vi "RemoteVI Accept Clients.vi"(0 "new connection":u32, 1 "html":string, 2 "hello":string, 3 "overlay frame":string, 5 "accepted?":bool, 7 "pending":T2(array[cluster]), 8 "new address":string, 9 "clients":T1(array[cluster]), 10 "token":string, 11 "view only?":bool, 12 "hWnd":u64) -> (4 "pending out":T2(array[cluster]), 6 "clients out":T1(array[cluster]))   [LabVIEW 2020, in "RemoteVI.lvlib"]
doc: "Turns accepted TCP connections into WebSocket clients WITHOUT blocking the server loop. A connection accepted in this iteration (accepted? TRUE) joins pending with an empty head and the current tick count. Then every pending connection gets one step of RemoteVI Serve Pending Connection.vi: whatever has arrived of its request head is read with timeout 0; a complete head is answered (RemoteVI Handle Connection.vi - 503 for an upgrade while 8 clients are connected), and an upgraded connection is greeted and added to clients (RemoteVI Add Client.vi); a connection that is gone or has sent no complete head within 5 s is closed; the rest stay pending. So an idle connection - a browser's speculative preconnect - costs one zero-timeout read per iteration instead of stalling the loop. Connections are TCP refnums type-cast to U32."
uses:
  RemoteVI.lvlib
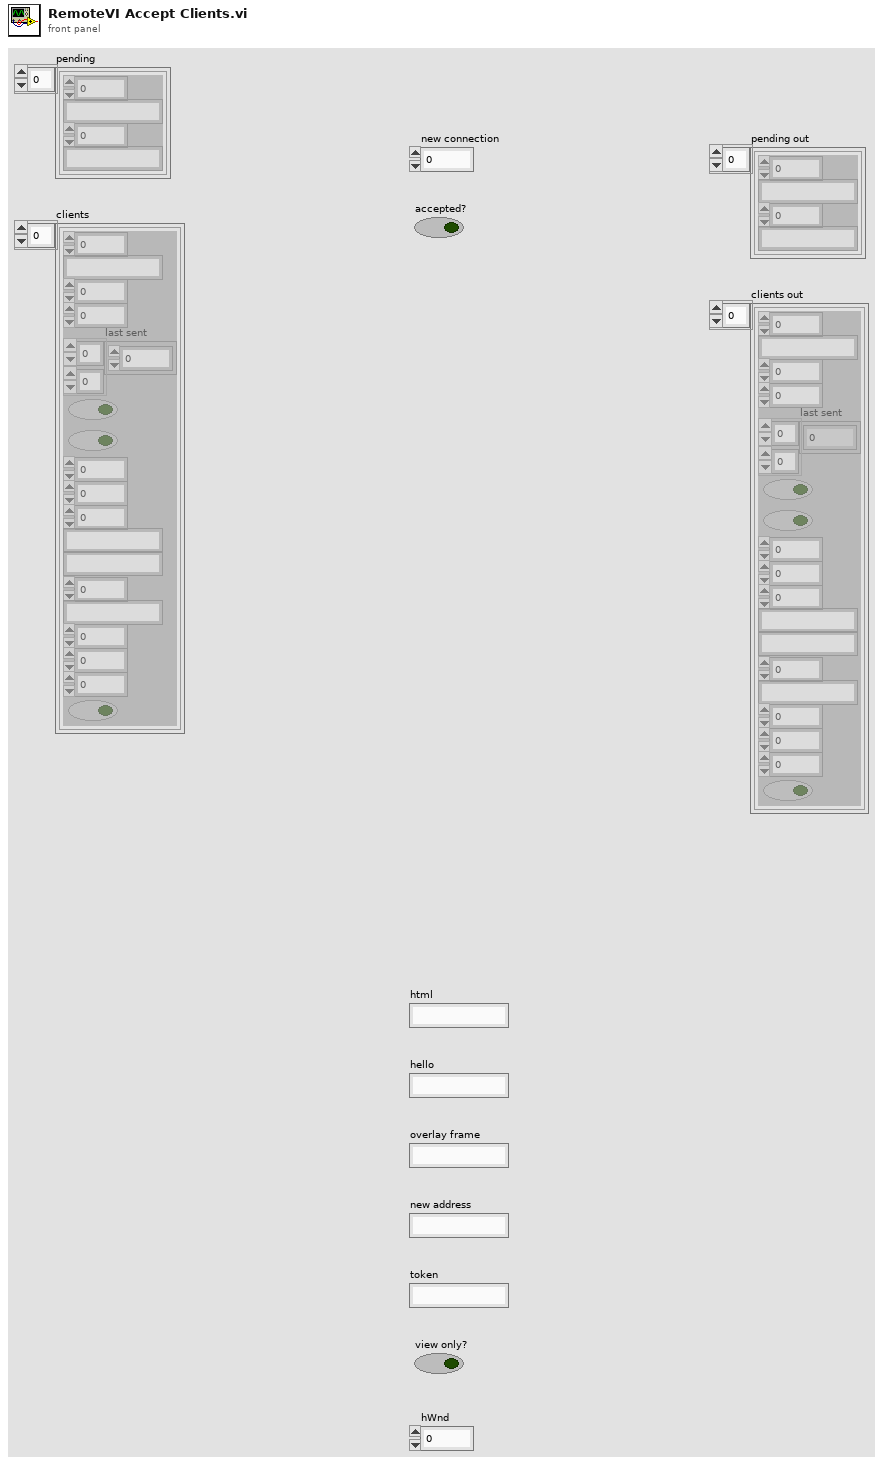
[diagram p1: front panel]
types:
  T1 = cluster{"connection":u32, "rx buffer":string, "seq":u32, "acked":u32, "last sent":u32[][], "tracking":bool, "closed":bool, "mods":u8, "mods set":u8, "popup since":u32, "windows sent":string, "window frames":cluster{"id":u64, "pixels":u32[][]}[], "key window":u64, "address":string, "since":dbl, "last input":dbl, "bytes":dbl, "view only":bool}[]
  T2 = cluster{"connection":u32, "head":string, "accepted":u32, "address":string}[]
  T3 = cluster{"connection":u32, "head":string, "accepted":u32, "address":string}
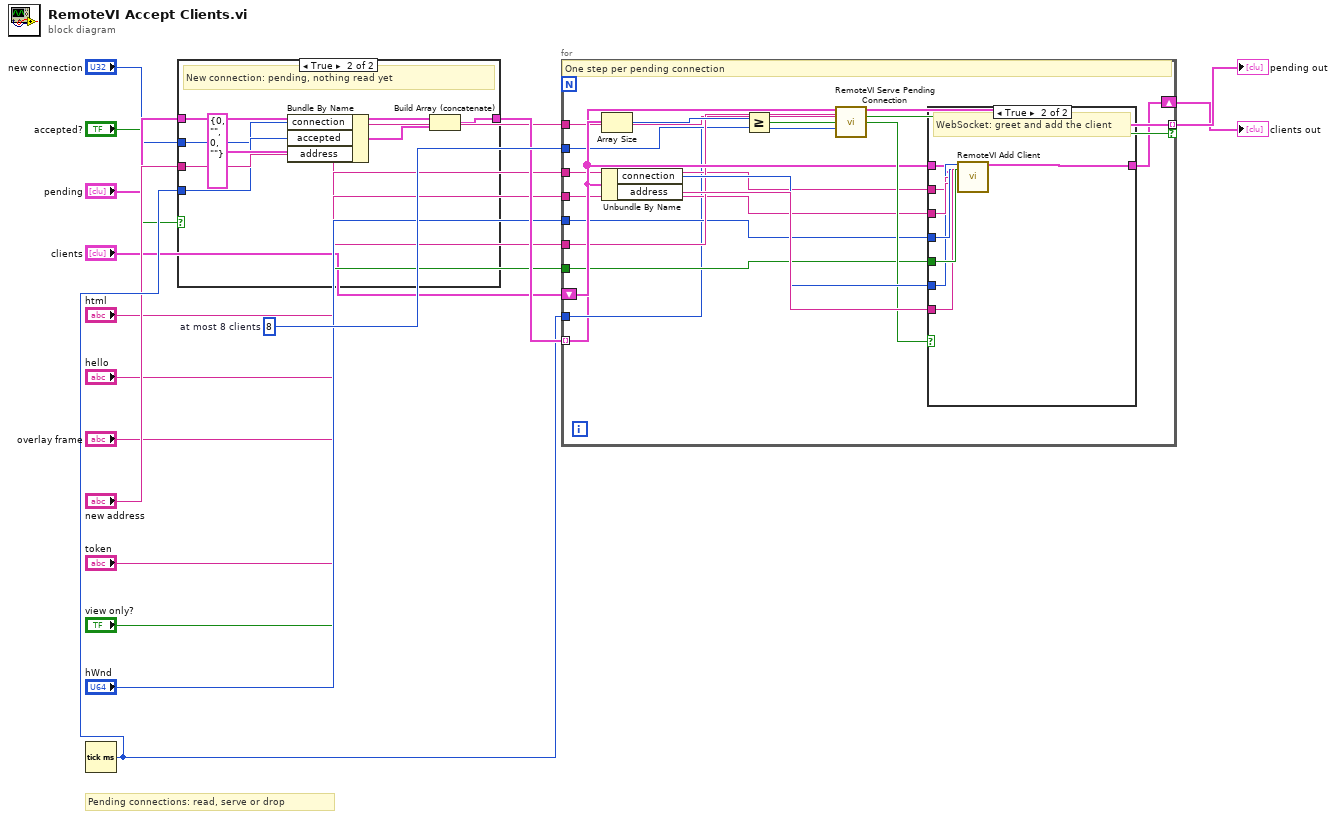
[diagram p0: block diagram]
diagram:
  w14 = 8  # at most 8 clients
  # "Pending connections: read, serve or drop"
  n1 = Tick Count (ms)() -> (millisecond timer value=w12:u32)
  n2 = case shown="True" "accepted?" {
    tunnel: "pending" -> [w17 w18]
    tunnel: "new connection" -> [_ w19]
    tunnel: "new address" -> [_ w21]
    tunnel: w12 -> [_ w20]
    tunnel: [w17 w24] -> w13
    frame False {
    }
    frame True {
      # "New connection: pending, nothing read yet"
      n3 = Bundle By Name(cluster=T3 {"connection"=0, "head"="", "accepted"=0, "address"=""}, "connection"=w19, "accepted"=w20, "address"=w21) -> (w23:T3)
      n4 = Build Array (concatenate)(w18, w23) -> (w24:T2)
    }
  }
  n5 = for {
    tunnel: "html" -> [w26]
    tunnel: w14 -> [w28]
    tunnel: "hello" -> [w29]
    tunnel: "overlay frame" -> [w30]
    tunnel: "hWnd" -> [w31]
    tunnel: "token" -> [w32]
    tunnel: "view only?" -> [w33]
    shift-right: [w35] -> w15
    shift-left: "clients" -> [w34]
    tunnel: w12 -> [w27]
    tunnel: w13 -> [w25] mode=indexing
    tunnel: [w38] -> w16 mode=indexing if=w39
    # "One step per pending connection"
    n6 = Array Size(array=w34) -> (size(s)=w36:i32)
    n7 = Unbundle By Name(w25) -> ("connection"=w41:u32, "address"=w42:string)
    n8 = Greater Or Equal?(x=w36, y=w28) -> (x >= y?=w37:bool)
    n9 = call "RemoteVI Serve Pending Connection.vi"("pending"=w25, "token"=w32, "html"=w26, "max clients reached?"=w37, "now"=w27) -> ("pending out"=w38:T3, "keep?"=w39:bool, "websocket?"=w40:bool)  [unwired: 8 in]
    n10 = case shown="True" w40 {
      tunnel: w34 -> [w43 w44]
      tunnel: w29 -> [_ w46]
      tunnel: w30 -> [_ w47]
      tunnel: w31 -> [_ w48]
      tunnel: w33 -> [_ w50]
      tunnel: w41 -> [_ w45]
      tunnel: w42 -> [_ w49]
      tunnel: [w43 w51] -> w35
      frame False {
      }
      frame True {
        # "WebSocket: greet and add the client"
        n11 = call "RemoteVI Add Client.vi"("connection"=w45, "hWnd"=w48, "address"=w49, "view only?"=w50, "clients"=w44, "hello"=w46, "overlay frame"=w47) -> ("clients out"=w51:T1)  [unwired: 8 in]
      }
    }
  }
  "pending out" <- w16
  "clients out" <- w15
